vi "Create RPC Method.vi"(8 "error in (no error)":errorcluster, 10 "rpc method parameters":T1, 11 "server class in":refnum<vi>) -> (0 "error out":errorcluster, 2 "newly created ?":bool, 3 "server class out":refnum<vi>)   [LabVIEW 2019, in "gRPC Template Creation Utility.lvlib"]
uses:
  gRPC Template Creation Utility.lvlib
  TypeDefs/RPC Method Parameters.ctl
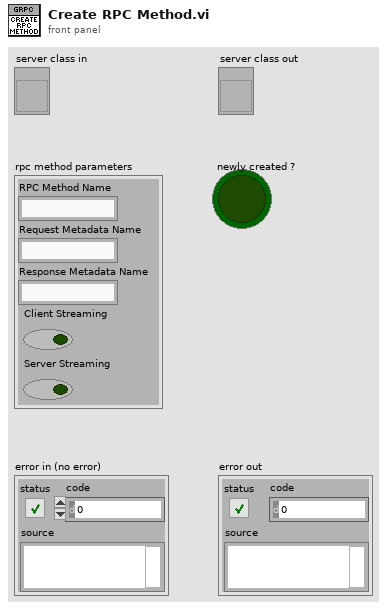
[diagram p1: front panel]
types:
  T1 = typedef "gRPC Template Creation Utility.lvlib/RPC Method Parameters.ctl" = cluster{"RPC Method Name":string, "Request Metadata Name":string, "Response Metadata Name":string, "Client Streaming":bool, "Server Streaming":bool}
  T2 = enum32{"invalid VI type", "Standard VI", "Control VI", "Global VI", "Polymorphic VI", "Configuration VI", "SubSystem", "Facade VI", "Method VI"}
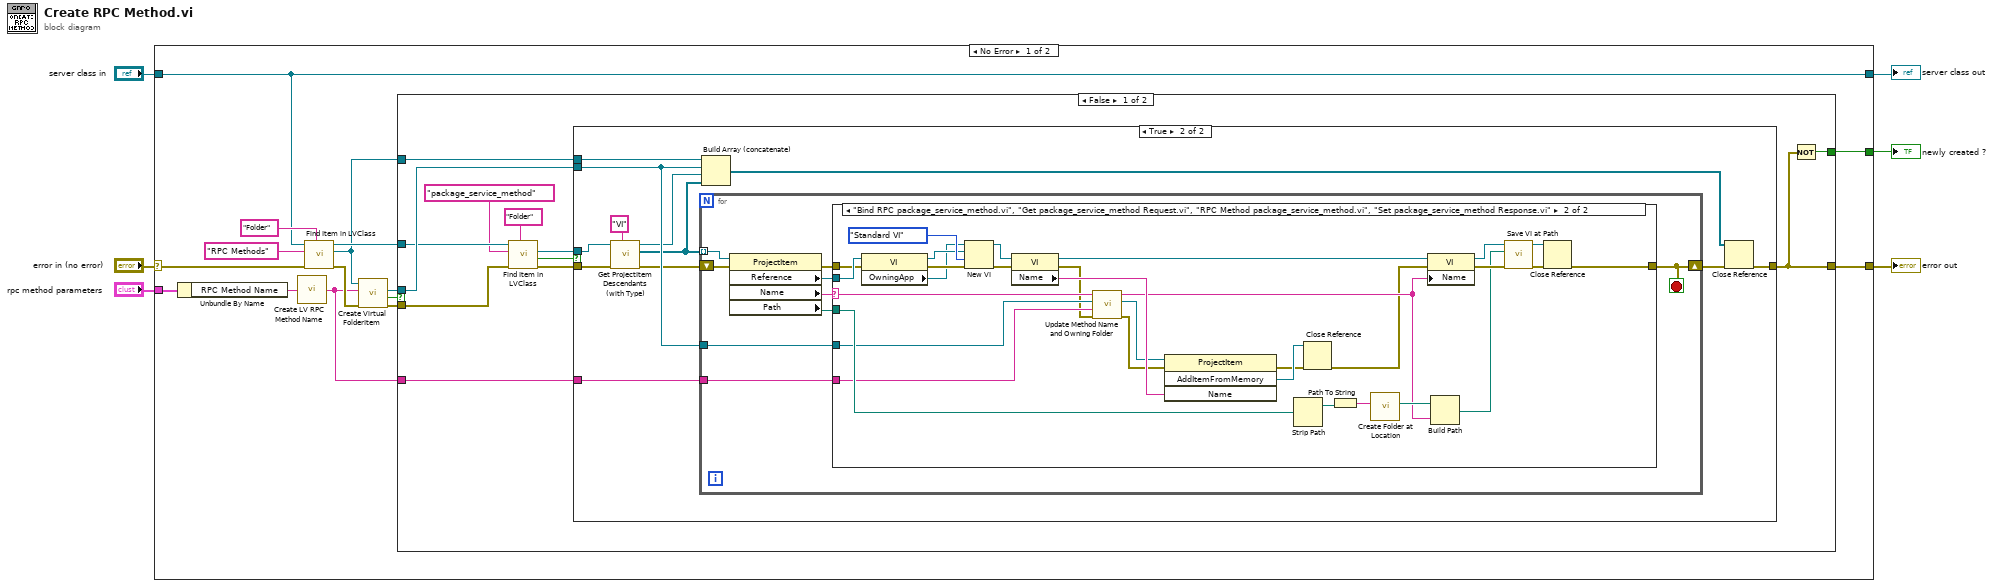
[diagram p0: block diagram]
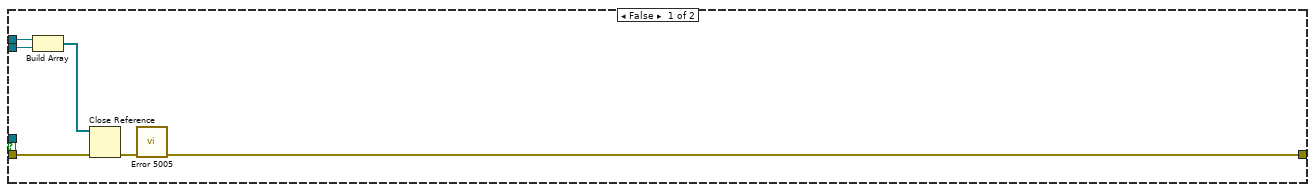
[diagram p2: hidden frame]
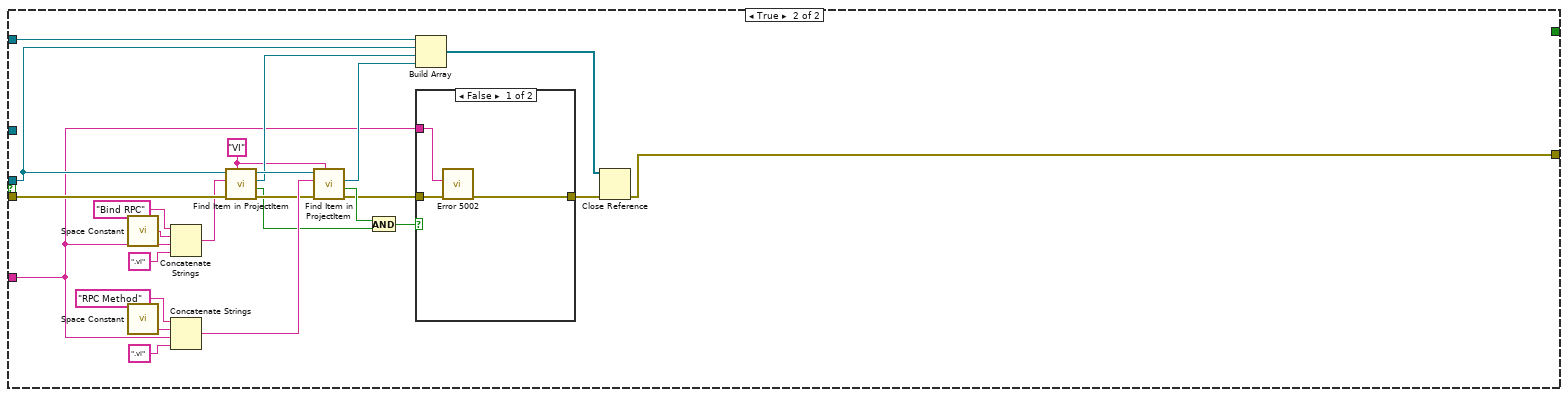
[diagram p4: hidden frame]
diagram:
  n1 = case shown="No Error" "error in (no error)" {
    selector: "error in (no error)" -> [w12 w121]
    tunnel: "server class in" -> [w11 w120]
    tunnel: [w17 w121] -> w5
    tunnel: [w11 w120] -> w3
    tunnel: [w10 _] -> w2
    tunnel: "rpc method parameters" -> [w9 _]
    frame No Error {
      n2 = Unbundle By Name(w9) -> ("RPC Method Name"=w8:string)
      n3 = call "Create LV RPC Method Name.vi"("Proto Parser RPC Method Name in"=w8) -> ("LV RPC Method Name out"=w7:string)
      n4 = call "Find Item in LVClass.vi"("Item Type"="Folder", "error in (no error)"=w12, "Item Name"="RPC Methods", "Class Item in"=w11) -> ("error out"=w16:errorcluster, "Project Item (Class Item)"=w14:refnum<vi>, "Class Item out"=w18:refnum<vi>)  [unwired: 4 in, 1 out]
      n5 = call "Create Virtual FolderItem.vi"("error in (no error)"=w16, "Folder Name"=w7, "ProjectItem in"=w14) -> ("error out"=w15:errorcluster, "Already exists?"=w21:bool, "FolderItem reference out"=w13:refnum<vi>)  [unwired: 5 in, 1 out]
      n6 = case shown="False" w21 {
        tunnel: w13 -> [w33 w100]
        tunnel: w14 -> [w32 w101]
        tunnel: w15 -> [w31 w115]
        tunnel: [w26 w92] -> w17
        tunnel: w18 -> [w30 _]
        tunnel: w7 -> [w27 w96]
        tunnel: [w25 _] -> w10
        frame False {
          n7 = call "Find Item in LVClass.vi"("Item Type"="Folder", "error in (no error)"=w31, "Item Name"="package_service_method", "Class Item in"=w30) -> ("error out"=w23:errorcluster, "Found?"=w22:bool, "Project Item (Class Item)"=w24:refnum<vi>)  [unwired: 4 in, 1 out]
          n8 = case shown="True" w22 {
            tunnel: w33 -> [w37 w51]
            tunnel: w32 -> [w38 w50]
            tunnel: w27 -> [_ w48]
            tunnel: [w39 w47] -> w26
            tunnel: w24 -> [_ w46]
            tunnel: w23 -> [w36 w45]
            frame False {
              n9 = Build Array(w38, w37) -> (w35:refnum<vi>[])
              n10 = Close Reference(reference=w35, error in (no error)=w36) -> (error out=w34:errorcluster)
              n11 = call "Error 5005.vi"("error in (no error)"=w34) -> ("error out"=w39:errorcluster)  [unwired: 10 in]
            }
            frame True {
              n12 = call "Get ProjectItem Descendants (with Type).vi"("Type"="VI", "error in (no error)"=w45, "ProjectItem in"=w46) -> ("error out"=w41:errorcluster, "All Descendents"=w42:refnum<vi>[], "ProjectItem out"=w43:refnum<vi>)  [unwired: 6 in]
              n13 = for {
                tunnel: w42 -> [w60] mode=indexing
                tunnel: w51 -> [w54]
                tunnel: w48 -> [w55]
                shift-right: [w52] -> w40
                shift-left: w41 -> [w59]
                stop <- w52 stop-if-true
                n14 = property class="ProjectItem"(reference=w60, error in=w59) -> (error out=w53:errorcluster, "Reference"=w57:refnum<vi>, "Name"=w58:string, "Path"=w56:path)  [unwired: 1 out]
                n15 = case shown="\"Bind RPC package_service_method.vi\", \"Get package_service_method Request.vi\", \"RPC Method package_service_method.vi\", \"Set package_service_method Response.vi\"" w58 {
                  selector: w58 -> [_ w74]
                  tunnel: w57 -> [_ w69]
                  tunnel: w56 -> [_ w77]
                  tunnel: w55 -> [_ w70]
                  tunnel: w54 -> [_ w72]
                  tunnel: w53 -> [w61 w67]
                  tunnel: [w61 w76] -> w52
                  frame "None", Default {
                  }
                  frame "Bind RPC package_service_method.vi", "Get package_service_method Request.vi", "RPC Method package_service_method.vi", "Set package_service_method Response.vi" {
                    n16 = property class="VI"(reference=w69, error in=w67) -> (reference out=w68:refnum<vi>, error out=w66:errorcluster, "OwningApp"=w65:refnum<vi>)
                    n17 = New VI(8:w66, 9:T2."Standard VI" ("vi type (standard vi)"), 10:w68, 11:w65) -> (0:w87:errorcluster, 3:w90:refnum<vi>)  [unwired: 3 out]
                    n18 = property class="VI"(reference=w90, error in=w87) -> (reference out=w88:refnum<vi>, error out=w64:errorcluster, "Name"=w91:string)
                    n19 = call "Update Method Name and Owning Folder.vi"("error in"=w64, "rpc method name"=w70, "rpc method folder"=w72, "original vi name"=w74) -> ("error out"=w63:errorcluster, "owning folder"=w71:refnum<vi>, "new vi name"=w73:string)  [unwired: 5 in]
                    n20 = invoke class="ProjectItem" method="AddItemFromMemory"(reference=w71, error in=w63, "Name"=w91) -> (error out=w78:errorcluster, "AddItemFromMemory"=w79:refnum<vi>)  [unwired: 1 in, 2 out]
                    n21 = Strip Path(path=w77) -> (stripped path=w75:path)  [unwired: 1 out]
                    n22 = Close Reference(reference=w79, error in (no error)=w78) -> (error out=w62:errorcluster)
                    n23 = Path To String(path=w75) -> (string=w84:string)
                    n24 = call "Create Folder at Location.vi"("Path"=w84) -> ("Full path out"=w83:path)  [unwired: 8 in, 2 out]
                    n25 = property class="VI"(reference=w88, error in=w62, "Name"=w73) -> (reference out=w86:refnum<vi>, error out=w85:errorcluster)
                    n26 = Build Path(base path=w83, name or relative path=w73) -> (appended path=w82:path)
                    n27 = call "Save VI at Path.vi"("error in (no error)"=w85, "Path"=w82, "VI in"=w86) -> ("error out"=w81:errorcluster, "VI out"=w80:refnum<vi>)  [unwired: 6 in, 1 out]
                    n28 = Close Reference(reference=w80, error in (no error)=w81) -> (error out=w76:errorcluster)
                  }
                }
              }
              n29 = Build Array (concatenate)(w50, w51, w43, w42) -> (w49:refnum<vi>[])
              n30 = Close Reference(reference=w49, error in (no error)=w40) -> (error out=w47:errorcluster)
            }
          }
          n31 = Not(x=w26) -> (.not. x?=w25:bool)
        }
        frame True {
          w94 = "VI" ("Type")
          n32 = call <vilib>:"Space Constant.vi"() -> ("String"=w109:string)
          n33 = call <vilib>:"Space Constant.vi"() -> ("String"=w108:string)
          n34 = Concatenate Strings("Bind RPC" ("string"), w109, w96, ".vi" ("string")) -> (w112:string)
          n35 = Concatenate Strings("RPC Method" ("string"), w108, w96, ".vi" ("string")) -> (w106:string)
          n36 = call "Find Item in ProjectItem.vi"("Item Type"=w94, "error in (no error)"=w115, "Name"=w112, "ProjectItem in"=w100) -> ("error out"=w105:errorcluster, "Found ?"=w104:bool, "Item Refnum out"=w99:refnum<vi>, "ProjectItem out"=w114:refnum<vi>)  [unwired: 4 in]
          n37 = call "Find Item in ProjectItem.vi"("Item Type"=w94, "error in (no error)"=w105, "Name"=w106, "ProjectItem in"=w114) -> ("error out"=w97:errorcluster, "Found ?"=w103:bool, "Item Refnum out"=w98:refnum<vi>)  [unwired: 4 in, 1 out]
          n38 = And(x=w103, y=w104) -> (x .and. y?=w102:bool)
          n39 = Build Array(w101, w100, w99, w98) -> (w95:refnum<vi>[])
          n40 = case shown="False" w102 {
            tunnel: w97 -> [w118 w119]
            tunnel: w96 -> [w116 _]
            tunnel: [w117 w119] -> w93
            frame False {
              n41 = call "Error 5002.vi"("error in (no error)"=w118, "Method Name"=w116) -> ("error out"=w117:errorcluster)  [unwired: 9 in]
            }
            frame True {
            }
          }
          n42 = Close Reference(reference=w95, error in (no error)=w93) -> (error out=w92:errorcluster)
        }
      }
    }
    frame Error {
    }
  }
  "error out" <- w5
  "server class out" <- w3
  "newly created ?" <- w2
